vi "CSM MDI.vi"(7 "Name (\"\" to Use UUID)":string="Event CSM") -> ()   [LabVIEW 2020, in "MDI ViewManager.lvlib"]
uses:
  MDI ViewManager.lvlib
  Typedef/View.ctl
  <vilib>/Utility/miscctls.llb/LVPointTypeDef.ctl
  <vilib>/Utility/miscctls.llb/LVPoint32TypeDef.ctl
  Typedef/Layout.ctl
  <vilib>/Utility/miscctls.llb/LVBoundsTypeDef.ctl
  <vilib>/Utility/miscctls.llb/LVPositionTypeDef.ctl
  <vilib>/Utility/miscctls.llb/LVRectTypeDef.ctl
  Typedef/Update View.ctl
  49dae65a-a1df-4644-8631-e10cd2ecf887.vi
  81b46446-0aca-48f9-86dc-ebdbbb8ef4b6.vi
  7ba8cf38-d999-4af7-9cb2-e6092c4454ab.vi
  5110686f-90b8-48a6-8112-abce107b1655.vi
  <userlib>/_NEVSTOP/Communicable State Machine(CSM)/AdvanceAPI/CSM - Revert Arguments-Safe String.vi
  <userlib>/_NEVSTOP/Communicable State Machine(CSM)/_Shared/Trim Single-line Text.vi
  <userlib>/_NEVSTOP/Communicable State Machine(CSM)/AdvanceAPI/CSM - Make String Arguments Safe.vi
  <userlib>/_NEVSTOP/Communicable State Machine(CSM)/AdvanceAPI/CSM - Break Down Multiple States String.vi
  <userlib>/_NEVSTOP/Communicable State Machine(CSM)/AdvanceAPI/CSM - Compact Multiple States.vi
  49dae65a-a1df-4644-8631-e10cd2ecf887.vi/b09b9099-6be0-413b-8afc-4908471460c3.vi
  <userlib>/_NEVSTOP/Communicable State Machine(CSM)/addons/INI-Static-Variable-Support/_Support/FlagInstance-CSMINIVariable.vi
  81b46446-0aca-48f9-86dc-ebdbbb8ef4b6.vi/99de0c97-112a-4c86-9094-c187659127e1.vi
  <userlib>/_NEVSTOP/Communicable State Machine(CSM)/AdvanceAPI/CSM - Keywords.vi
  <userlib>/_NEVSTOP/Communicable State Machine(CSM)/_Support/ChangeFlag/ChangeFlag-Read.vi
  <userlib>/_NEVSTOP/Communicable State Machine(CSM)/_Support/ChangeFlag/ChangeFlagDB.vi
  <vilib>/Utility/Data Type/Get Type Information.vi
  <userlib>/_NEVSTOP/Communicable State Machine(CSM)/addons/API-String-Arugments-Support/_Support/Data To SingleElementsArray_csm.vi
  <userlib>/_NEVSTOP/Communicable State Machine(CSM)/addons/INI-Static-Variable-Support/_Support/Parse Used Session and Name.vi
  <userlib>/_NEVSTOP/Communicable State Machine(CSM)/addons/API-String-Arugments-Support/_Support/Data To API String Arguments.vi
  <userlib>/_NEVSTOP/Communicable State Machine(CSM)/addons/INI-Static-Variable-Support/_Support/INI-FGV(lvlibp).vi
  <userlib>/_NEVSTOP/Communicable State Machine(CSM)/addons/INI-Static-Variable-Support/_Support/Populate String with INI Variable.vi
  <userlib>/_NEVSTOP/Communicable State Machine(CSM)/addons/API-String-Arugments-Support/_Support/Convert API String Arguments to Data(variant).vi
  <userlib>/_NEVSTOP/Communicable State Machine(CSM)/addons/API-String-Arugments-Support/_Support/SingleElementsArray To Data_csm.vi
  <userlib>/_NEVSTOP/Communicable State Machine(CSM)/Communicable State Machine.lvlib
  <userlib>/_NEVSTOP/Communicable State Machine(CSM)/addons/INI-Static-Variable-Support/INI-Static-Variable-Support.lvlib
panel:
  in  "Tab Control 40":T1 caption="View0"
  in  "Tab Control 39":T1 caption="View1"
  in  "Tab Control 38":T1 caption="View2"
  in  "Tab Control 37":T1 caption="View3"
  in  "Tab Control 36":T1 caption="View4"
  in  "Tab Control 35":T1 caption="View5"
  in  "Tab Control 34":T1 caption="View6"
  in  "Tab Control 33":T1 caption="View7"
  in  "Tab Control 32":T1 caption="View8"
  in  "Tab Control 31":T1 caption="View9"
  in  "Tab Control 30":T1 caption="View10"
  in  "Tab Control 29":T1 caption="View11"
  in  "Tab Control 28":T1 caption="View12"
  in  "Tab Control 27":T1 caption="View13"
  in  "Tab Control 26":T1 caption="View14"
  in  "Tab Control 25":T1 caption="View15"
  in  "Tab Control 24":T1 caption="View16"
  in  "Tab Control 23":T1 caption="View17"
  in  "Tab Control 22":T1 caption="View18"
  in  "Tab Control 21":T1 caption="View19"
  in  "Tab Control 20":T1 caption="View20"
  in  "Tab Control 19":T1 caption="View21"
  in  "Tab Control 18":T1 caption="View22"
  in  "Tab Control 17":T1 caption="View23"
  in  "Tab Control 16":T1 caption="View24"
  in  "Tab Control 15":T1 caption="View25"
  in  "Tab Control 14":T1 caption="View26"
  in  "Tab Control 13":T1 caption="View27"
  in  "Tab Control 12":T1 caption="View28"
  in  "Tab Control 11":T1 caption="View29"
  in  "Tab Control 10":T1 caption="View30"
  in  "Tab Control 9":T1 caption="View31"
  in  "Tab Control 8":T1 caption="View32"
  in  "Tab Control 7":T1 caption="View33"
  in  "Tab Control 6":T1 caption="View34"
  in  "Tab Control 5":T1 caption="View35"
  in  "Tab Control 4":T1 caption="View36"
  in  "Tab Control 3":T1 caption="View37"
  in  "Tab Control 2":T1 caption="View38"
  in  "Tab Control":T1 caption="View39"
  out "State History":string
types:
  T1 = typedef "MDI ViewManager.lvlib/View.ctl" = enum32{"Page 1", "Page 2"}
  T2 = typedef "LVPointTypeDef.ctl" = cluster{"Horizontal":i16, "Vertical":i16}
  T3 = typedef "LVPoint32TypeDef.ctl" = cluster{"Horizontal":i32, "Vertical":i32}
  T4 = typedef "MDI ViewManager.lvlib/Layout.ctl" = cluster{"Origin":T2, "Layout":cluster{"Pane Dimension":T5, "Position":T6, "Label":string, "Visible":bool, "InsertedViewName":string}[], "Horizontal Scrollbar Visibility":enum16{"Always On", "Always Off", "Off While Running"}, "Vertical Scrollbar Visibility":enum16{"Always On", "Always Off", "Off While Running"}, "Position":T6, "Rect":T7}
  T5 = typedef "LVBoundsTypeDef.ctl" = cluster{"Width":u32, "Height":u32}
  T6 = typedef "LVPositionTypeDef.ctl" = cluster{"Left":i32, "Top":i32}
  T7 = typedef "LVRectTypeDef.ctl" = cluster{"Left":i16, "Top":i16, "Right":i16, "Bottom":i16}
  T8 = typedef "MDI ViewManager.lvlib/Update View.ctl" = cluster{"Name":string, "VIPath":path, "Height(Default)":u32, "Widht(Default)":u32, "VIRef":refnum<vi>}
  T9 = cluster{"Ref":cluster{"TabCtls":refnum<vi>[], "CurrMoveCtl":refnum<vi>, "Pane":refnum<vi>, "SubPanel":refnum<vi>, "Caller VI":refnum<vi>}, "Val":cluster{"TabCtlMove?":bool, "MouseOffset":T3, "LayoutMap":map{string, T4}, "ViewMap":map{string, T8}, "Edit Mode?":bool}}
  T10 = cluster{"Current VI Reference":refnum<vi>, "Close Panel on Exit?":bool}
  T11 = cluster{"Core":cluster{"Current VI Reference":refnum<vi>, "Close Panel on Exit?":bool}, "1":cluster{"Ref":cluster{"TabCtls":refnum<vi>[], "CurrMoveCtl":refnum<vi>, "Pane":refnum<vi>, "SubPanel":refnum<vi>, "Caller VI":refnum<vi>}, "Val":cluster{"TabCtlMove?":bool, "MouseOffset":T3, "LayoutMap":map{string, T4}, "ViewMap":map{string, T8}, "Edit Mode?":bool}}}
  T12 = enum16{"Always On", "Always Off", "Off While Running"}
  T13 = enum32{"Invalid", "Standard", "Closed", "Hidden", "Minimized", "Maximized"}
  T14 = enum32{"invalid app kind", "Development System", "Run Time System", "Student Edition", "Embedded LabVIEW", "Evaluation", "Custom"}
  T15 = cluster{"TabCtl":refnum<vi>[], "Pane":refnum<vi>, "Variant":variant, "map in":map{string, T4}, "1.Ref.Caller VI":refnum<vi>}
  T16 = cluster{"Pane":refnum<vi>, "TabCtls":refnum<vi>[], "Layout Map":map{string, T4}, "View Map":map{string, T8}, "1.Ref.Caller VI":refnum<vi>}
  T17 = typedef "Communicable State Machine.lvlib/_CSM_Response Source Message.ctl" = cluster{"‘State":string, "’Arguments":string, "’Error":errorcluster}
  T18 = cluster{"TabCtlMove?":bool, "Caller VI":refnum<vi>, "CtlRef":refnum<vi>, "Double Click":bool, "Coords":T3, "Ctrl":bool}
  T19 = cluster{"CtlRef":refnum<vi>, "Coords":T3, "TabCtlMove?":bool}
  T20 = cluster{"LayoutMap":map{string, T4}, "Edit Mode?":bool}
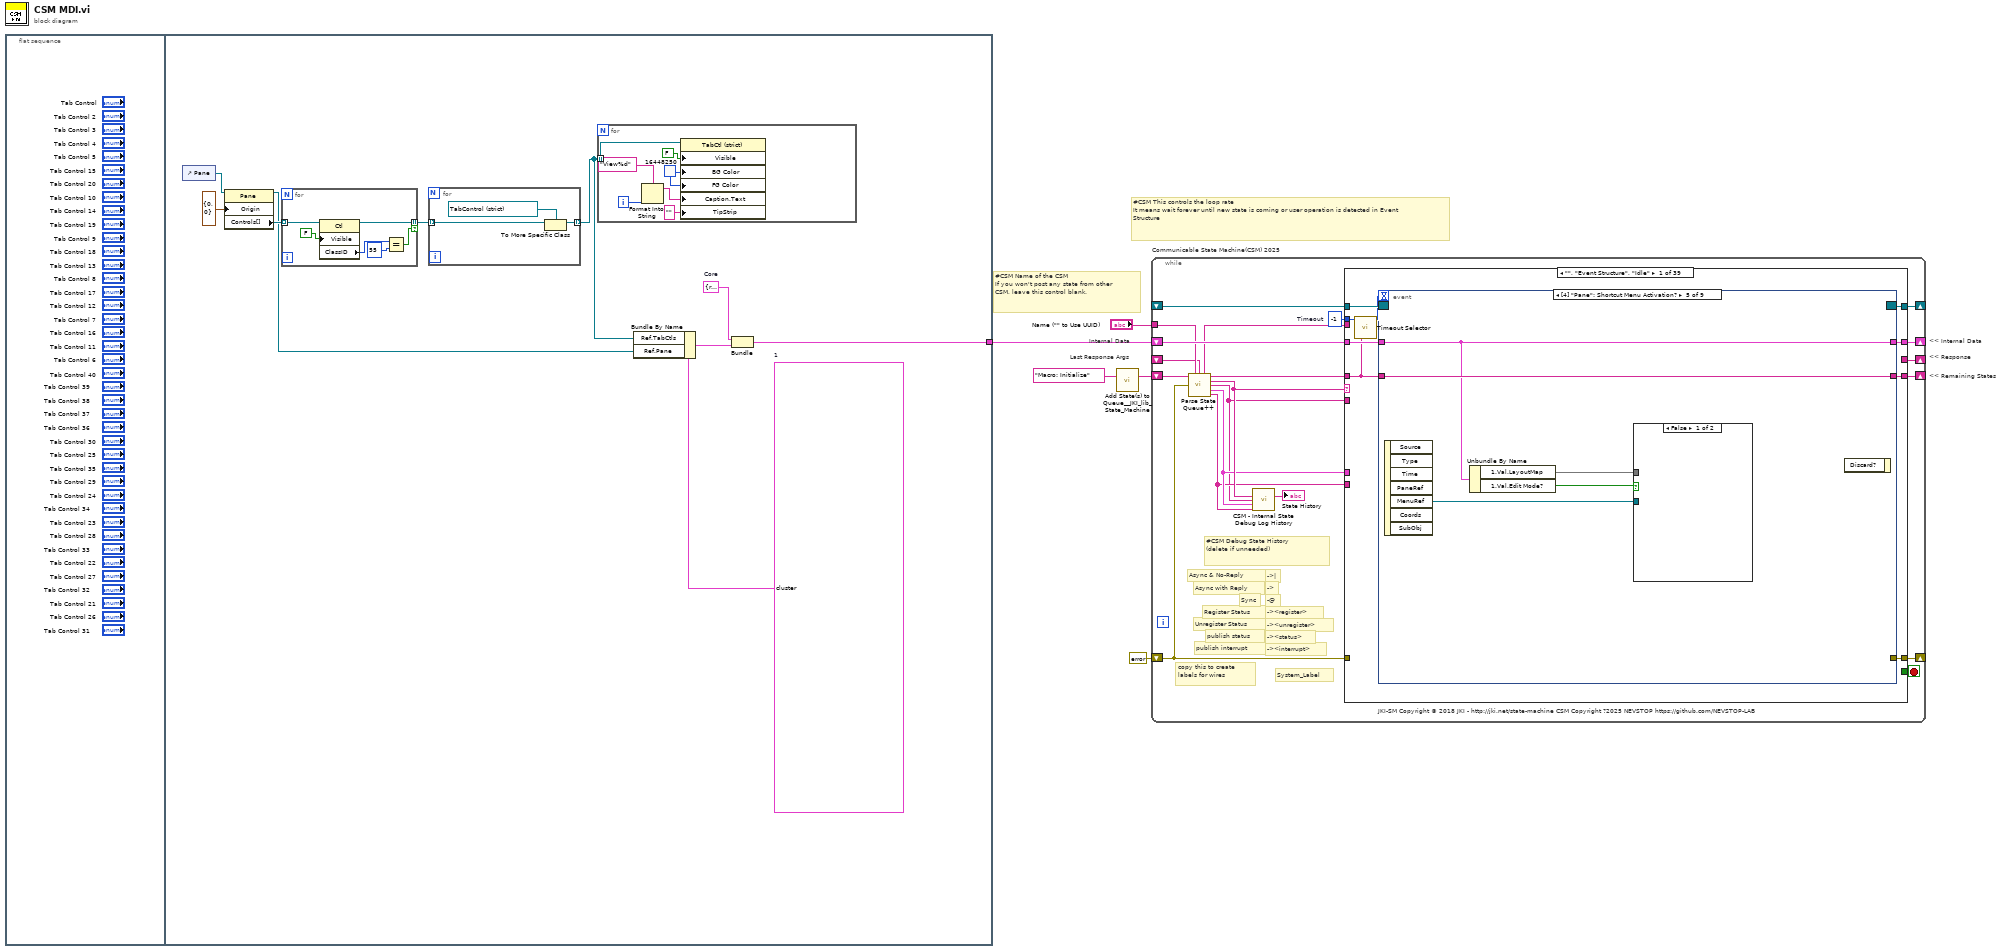
[diagram p0: block diagram]
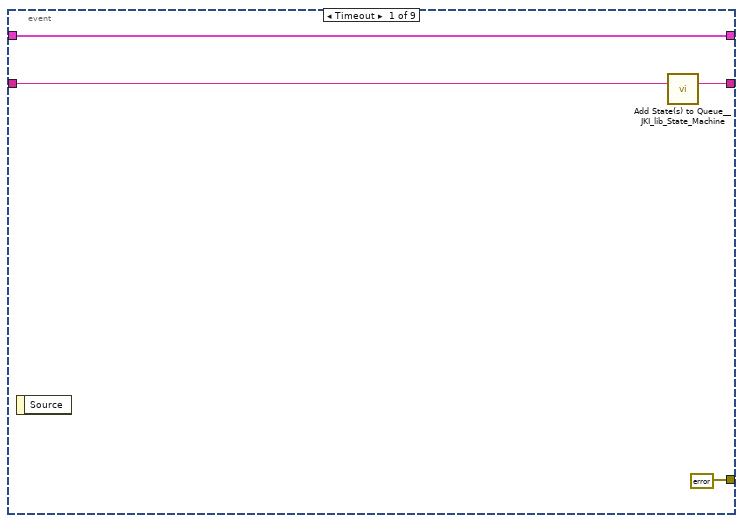
[diagram p2: hidden frame]
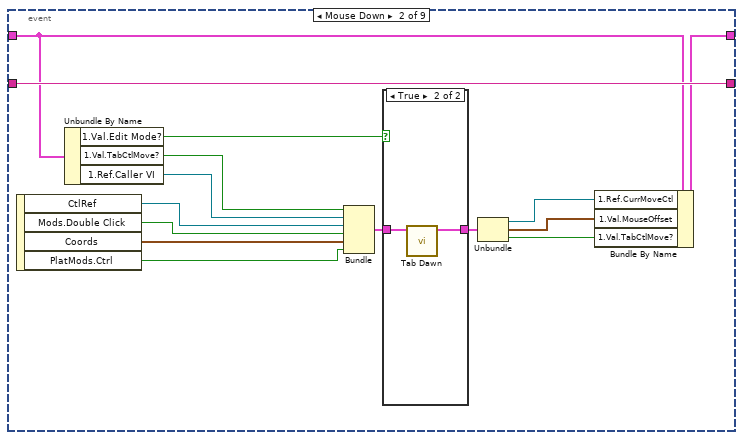
[diagram p3: hidden frame]
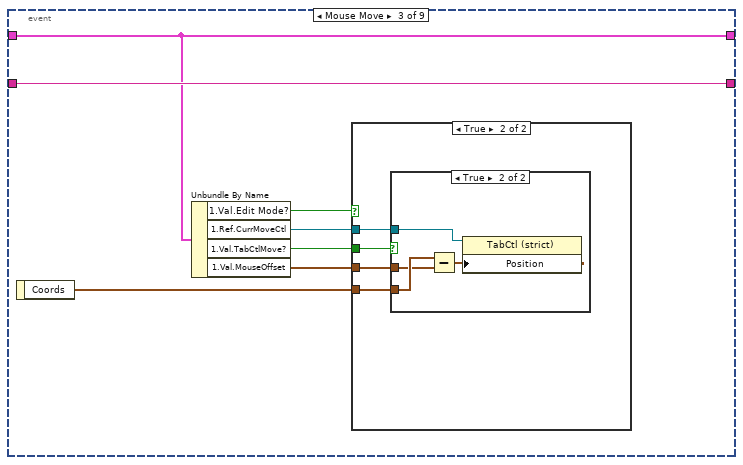
[diagram p5: hidden frame]
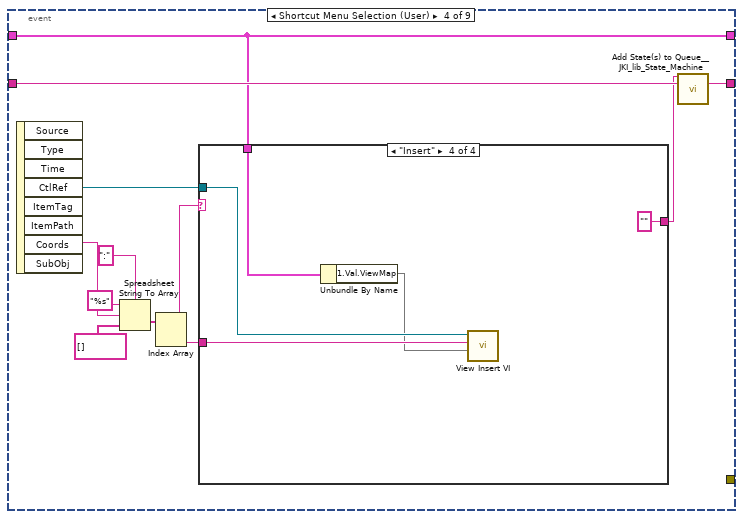
[diagram p8: hidden frame]
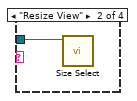
[diagram p10: hidden frame]
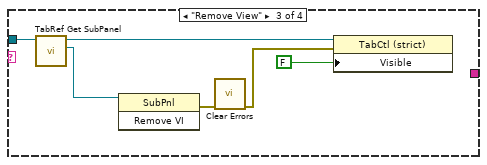
[diagram p11: hidden frame]
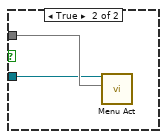
[diagram p12: hidden frame]
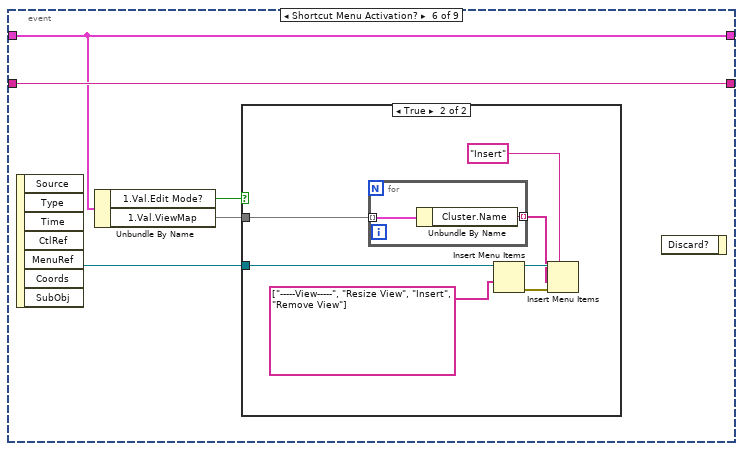
[diagram p13: hidden frame]
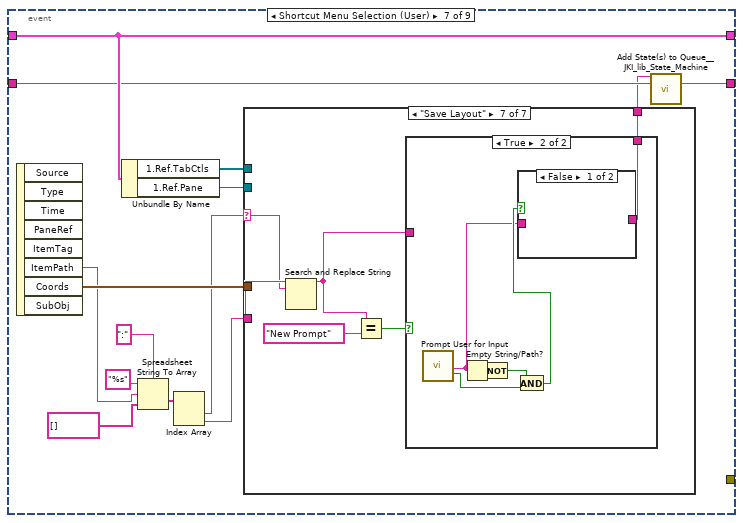
[diagram p15: hidden frame]
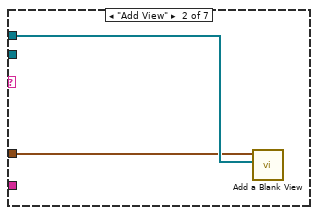
[diagram p17: hidden frame]
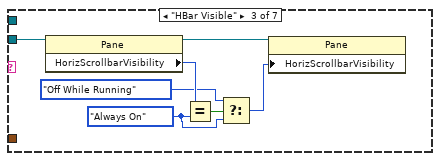
[diagram p18: hidden frame]
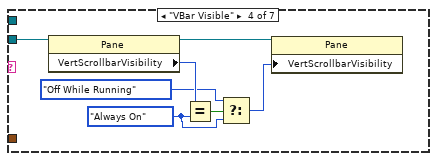
[diagram p19: hidden frame]
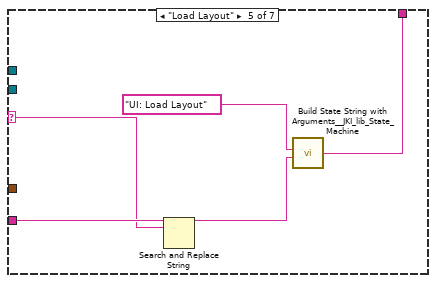
[diagram p20: hidden frame]
diagram:
  # "Last Response Args"
  # "Internal Data"
  # "<< Internal Data"
  # "<< Response"
  # "<< Remaining States"
  # "#CSM Name of the CSM\nIf you won't post any state from other CSM, leave this control blank."
  # "#CSM This controls the loop rate\nIt means wait forever until new state is coming or user operation is detected in Event Structure"
  n1 = flat-sequence {
    tunnel: [w15] -> w1
    frame #0 {
    }
    frame #1 {
      w13 = T9 {"Ref"={"TabCtls"=[], "CurrMoveCtl"=refnum, "Pane"=refnum, "SubPanel"=refnum, "Caller VI"=refnum}, "Val"={"TabCtlMove?"=FALSE, "MouseOffset"={"Horizontal"=0, "Vertical"=0}, "LayoutMap"={}, "ViewMap"={}, "Edit Mode?"=FALSE}}  # 1
      w12 = T10 {"Current VI Reference"=refnum, "Close Panel on Exit?"=FALSE}  # Core
      n2 = control-ref of="Pane"() -> (w6:refnum<vi>)
      n3 = property class="Pane"(reference=w6, "Origin"=T2 {"Horizontal"=0, "Vertical"=0}) -> (reference out=w7:refnum<vi>, "Controls[]"=w10:refnum<vi>[])  [unwired: 1 in, 1 out]
      n4 = for {
        tunnel: w10 -> [w24] mode=indexing
        tunnel: [w19] -> w9 mode=indexing if=w20
        n5 = property class="Ctl"(reference=w24, "Visible"=FALSE) -> (reference out=w19:refnum<vi>, "ClassID"=w22:u32)  [unwired: 1 in, 1 out]
        n6 = Equal?(x=w22, y=u32 55) -> (x = y?=w20:bool)
      }
      n7 = for {
        tunnel: w9 -> [w18] mode=indexing
        tunnel: [w17] -> w8 mode=indexing
        n8 = To More Specific Class(target class=refnum<vi> refnum ("Tab Control"), reference=w18) -> (specific class reference=w17:refnum<vi>)  [unwired: 1 in, 1 out]
      }
      n9 = for {
        tunnel: w8 -> [w30] mode=indexing
        i -> [w28]
        w29 = u32 16448250 ("Colors:BG Color")
        n10 = Format Into String(format string="View%d", w28) -> (resulting string=w27:string)  [unwired: 2 in, 1 out]
        n11 = property class="TabCtl (strict)"(reference=w30, "Visible"=FALSE, "BG Color"=w29, "FG Color"=w29, "Caption.Text"=w27, "TipStrip"="" ("Tip Strip")) -> ()  [unwired: 1 in, 2 out]
      }
      n12 = Bundle By Name(cluster=w13, "Ref.TabCtls"=w8, "Ref.Pane"=w7) -> (w14:T9)
      n13 = Bundle("Core"=w12, "1"=w14) -> (w15:T11)  [unwired: 1 in]
    }
  }
  n14 = call <vilib>:"Add State(s) to Queue__JKI_lib_State_Machine.vi"("State(s) in (\"\")"="Macro: Initialize" ("Init State(\"Macro: Initialize\")")) -> ("States Out"=w2:string)  [unwired: 14 in]
  n15 = while "Communicable State Machine(CSM) 2025" {
    shift-right: [w46] -> _
    shift-left: w1 -> [w45]
    shift-right: [w49] -> _
    shift-left: errorcluster {"status"=FALSE, "code"=0, "source"=""} ("error out") -> [w43]
    shift-right: [w48] -> _
    shift-left: w2 -> [w50]
    tunnel: "Name (\"\" to Use UUID)" -> [w39]
    shift-right: [w42] -> _
    shift-left: _ -> [w34]
    shift-right: [w41] -> _
    shift-left: _ -> [w40]
    stop <- w47 stop-if-true
    w44 = -1  # Timeout
    # "#CSM Debug State History\n(delete if unneeded)"
    # "-><interrupt>"
    # "-><status>"
    # "-><unregister>"
    # "-><register>"
    # "-@"
    # "->"
    # "->|"
    # "publish interrupt"
    # "publish status"
    # "Unregister Status"
    # "Register Status"
    # "Sync"
    # "Async with Reply"
    # "Async & No-Reply"
    # "copy this to create labels for wires"
    # "System_Label"
    # "JKI-SM Copyright © 2018 JKI - http://jki.net/state-machine CSM Copyright ?2025 NEVSTOP https://github.com/NEVSTOP-LAB"
    n16 = call <userlib>:"Parse State Queue++.vi"("State Queue"=w50, "Name (\"\" to Use UUID)"=w39, "Response Arguments"=w34, "Previous Error"=w43) -> ("Name Used"=w35:string, "Remaining States"=w51:string, "Current State"=w38:string, "Arguments"=w33:string, "Additional Information"=w37:T17, "Source CSM"=w36:string)  [unwired: 6 in]
    n17 = call <userlib>:"CSM - Internal State Debug Log History.vi"("State"=w38, "Arguments (\"\")"=w33, ">> Response Source Message >>"=w37, "Source (\"\")"=w36) -> ("Debug Log"=→"State History":string)  [unwired: 11 in]
    n18 = case shown="\"\", \"Event Structure\", \"Idle\"" w38 {
      selector: w38 -> [_ _ _ w223 _ _ _ _ _ _ _ _ _ _ _ _ _ _ _ _ _ _ _ _ _ _ _ _ _ _ _ _ _ _ _ _ _ _ _]
      tunnel: w51 -> [w53 w215 w220 w229 w235 w241 w267 w275 w282 w292 w301 w314 w319 w323 w329 w352 w356 w366 w370 w374 w378 w392 w412 w417 w428 w447 w458 w522 w535 w546 w549 w559 w561 w578 w586 w601 w606 w610 w614]
      tunnel: w33 -> [_ _ _ _ _ w239 w263 w270 w278 w286 _ _ _ _ _ _ _ _ _ _ _ w388 w407 w413 _ w443 w453 _ _ _ _ w550 w564 w579 w587 w597 _ _ _]
      tunnel: w45 -> [w59 w214 w217 w227 w234 w247 w268 w273 w280 w290 w300 w308 w317 w321 w326 w348 w354 w358 w369 w372 w375 w387 w410 w416 w429 w445 w455 w520 w523 w544 w548 w557 w572 w583 w591 w595 w604 w608 w612]
      tunnel: [w58 _ w218 w221 w236 errorcluster {"status"=FALSE, "code"=0, "source"=""} ("error out") w260 w269 w276 w289 _ _ _ _ _ w349 _ w361 w368 _ _ w389 w396 w418 w439 w444 w456 _ _ _ _ _ w563 w580 w588 w602 _ _ _] -> w49
      tunnel: w43 -> [_ _ w218 w222 w236 w245 w261 w271 w277 _ _ _ _ _ _ w345 _ _ _ _ _ w390 w401 w418 w439 _ _ _ _ _ _ _ w567 w580 w588 w602 _ _ _]
      tunnel: [w60 w215 w219 w228 w235 w243 w266 w274 w281 w293 w301 w313 w318 w322 w328 w351 w355 w366 w370 w373 w377 w392 w412 w417 w427 w446 w457 w521 w534 w545 w549 w559 w560 w577 w585 w601 w605 w609 w613] -> w48
      tunnel: [_ _ _ _ _ _ TRUE _ _ _ _ _ TRUE _ _ _ _ _ _ _ _ _ _ _ _ _ _ _ _ _ _ _ _ _ _ _ _ _ _] -> w47
      tunnel: [w57 w214 w217 w227 w234 w247 w268 w273 w280 w291 w300 w312 w317 w321 w325 w348 w354 w358 w369 w372 w375 w381 w410 w414 w429 w445 w455 w520 w523 w544 w548 w555 w570 w583 w591 w598 w604 w608 w612] -> w46
      tunnel: w44 -> [w55 _ _ _ _ _ _ _ _ _ _ _ _ _ _ _ _ _ _ _ _ _ _ _ _ _ _ _ _ _ _ _ _ _ _ _ _ _ _]
      tunnel: w36 -> [_ _ _ _ _ w238 _ _ _ w287 _ _ _ _ _ _ _ _ _ _ _ _ _ _ _ _ _ _ _ _ _ _ _ _ _ _ _ _ _]
      tunnel: w37 -> [_ _ _ _ _ w237 _ _ _ w288 _ _ _ _ _ _ _ _ _ _ _ _ _ _ _ _ _ _ _ _ _ _ _ _ _ _ _ _ _]
      tunnel: [_ _ _ "" w230 _ _ _ _ _ _ _ _ _ _ _ _ _ _ _ _ _ _ _ _ _ _ _ _ _ _ _ _ _ _ _ _ _ _] -> w42
      tunnel: [w52 w213 w216 w225 w233 w246 w264 w272 w279 w294 w299 w302 w315 w320 w327 w347 w353 w365 w367 w371 w376 w391 w411 w415 w438 w442 w452 w519 w533 w537 w547 w558 w575 w582 w590 w600 w603 w607 w611] -> w41
      tunnel: w40 -> [w56 w213 w216 w225 w233 w246 w264 w272 w279 w294 w299 w302 w315 w320 w327 w347 w353 _ w367 w371 w376 w391 w411 w415 w438 w442 w452 w519 w533 w537 w547 w558 w575 w582 w590 w600 w603 w607 w611]
      tunnel: w35 -> [_ _ _ w224 _ _ w262 _ _ _ _ _ _ _ w324 w343 _ w364 _ _ _ _ _ _ _ _ _ _ _ _ _ _ _ _ _ _ _ _ _]
      frame "", "Event Structure", "Idle" {
        n19 = call <userlib>:"Timeout Selector.vi"("Remaining States"=w53, "Timeout Expected"=w55) -> ("Timeout"=w54:i32)  [unwired: 5 in]
        n20 = event shown="[4] \"Pane\": Shortcut Menu Activation?" {
          selector: w56 -> [_ _ _ _ _ _ _ _ _]
          dyn-events: [_ _ _ _ _ _ _ _ _] -> w52
          timeout: w54 -> [_ _ _ _ _ _ _ _ _]
          tunnel: w53 -> [w64 w79 w88 w107 w125 w132 w153 w200 w212]
          tunnel: [w63 w79 w88 w106 w125 w132 w152 w200 w211] -> w60
          tunnel: w59 -> [w62 w78 w86 w97 w124 w131 w155 w201 w210]
          tunnel: [errorcluster {"status"=FALSE, "code"=0, "source"=""} ("error out") _ _ _ _ _ _ _ _] -> w58
          tunnel: [w62 w77 w86 w97 w124 w131 w155 w201 w210] -> w57
          event Timeout {
            n21 = event-data() -> ()  [unwired: 1 in, 1 out]
            n22 = call <vilib>:"Add State(s) to Queue__JKI_lib_State_Machine.vi"("State(s) in (\"\")"=w64) -> ("States Out"=w63:string)  [unwired: 14 in]
          }
          event Mouse Down {
            n23 = event-data() -> ("CtlRef"=w74:refnum<vi>, "Mods.Double Click"=w73:bool, "Coords"=w72:T3, "PlatMods.Ctrl"=w65:bool)  [unwired: 1 in]
            n24 = Unbundle By Name(w78) -> ("1.Val.Edit Mode?"=w66:bool, "1.Val.TabCtlMove?"=w76:bool, "1.Ref.Caller VI"=w75:refnum<vi>)
            n25 = Bundle("TabCtlMove?"=w76, "Caller VI"=w75, "CtlRef"=w74, "Double Click"=w73, "Coords"=w72, "Ctrl"=w65) -> (w71:T18)  [unwired: 1 in]
            n26 = case shown="True" w66 {
              tunnel: w71 -> [_ w81]
              tunnel: [_ w80] -> w70
              frame False {
              }
              frame True {
                n27 = call "Tab Dawn.vi"("output cluster"=w81) -> ("output cluster 2"=w80:T19)  [unwired: 10 in]
              }
            }
            n28 = Unbundle(w70) -> ("CtlRef"=w69:refnum<vi>, "Coords"=w68:T3, "TabCtlMove?"=w67:bool)
            n29 = Bundle By Name(cluster=w78, "1.Ref.CurrMoveCtl"=w69, "1.Val.MouseOffset"=w68, "1.Val.TabCtlMove?"=w67) -> (w77:T11)
          }
          event Mouse Move {
            n30 = event-data() -> ("Coords"=w87:T3)  [unwired: 1 in]
            n31 = Unbundle By Name(w86) -> ("1.Val.Edit Mode?"=w82:bool, "1.Ref.CurrMoveCtl"=w84:refnum<vi>, "1.Val.TabCtlMove?"=w85:bool, "1.Val.MouseOffset"=w83:T3)
            n32 = case shown="True" w82 {
              tunnel: w87 -> [_ w92]
              tunnel: w85 -> [_ w91]
              tunnel: w84 -> [_ w90]
              tunnel: w83 -> [_ w89]
              frame False {
              }
              frame True {
                n33 = case shown="True" w91 {
                  tunnel: w92 -> [_ w96]
                  tunnel: w90 -> [_ w95]
                  tunnel: w89 -> [_ w93]
                  frame False {
                  }
                  frame True {
                    n34 = Subtract(x=w96, y=w93) -> (x-y=w94:T3)
                    n35 = property class="TabCtl (strict)"(reference=w95, "Position"=w94) -> ()  [unwired: 1 in, 2 out]
                  }
                }
              }
            }
          }
          event Shortcut Menu Selection (User) {
            n36 = event-data() -> ("CtlRef"=w108:refnum<vi>, "ItemPath"=w103:string)  [unwired: 1 in, 6 out]
            n37 = Spreadsheet String To Array(delimiter (Tab)=":", format string="%s", spreadsheet string=w103, array type (2D Dbl)=string[] [] ("delimiter (Tab)")) -> (array=w100:string[])
            n38 = Index Array(array=w100) -> (element #1=w99:string, element #2=w98:string)  [unwired: 2 in]
            n39 = case shown="\"Insert\"" w99 {
              tunnel: w108 -> [_ w109 w115 w118]
              tunnel: [_ _ _ "" ("State(s) in Front (\"\")")] -> w105
              tunnel: w98 -> [_ _ _ w119]
              tunnel: w97 -> [_ _ _ w120]
              frame "False", Default {
              }
              frame "Resize View" {
                n40 = call "Size Select.vi"("CtlRef"=w109) -> ()  [unwired: 11 in]
              }
              frame "Remove View" {
                n41 = call "TabRef Get SubPanel.vi"("TabControl in"=w115) -> ("Sub Panel"=w111:refnum<vi>, "TabControl out"=w114:refnum<vi>)  [unwired: 8 in, 1 out]
                n42 = invoke class="SubPnl" method="Remove VI"(reference=w111) -> (error out=w112:errorcluster)  [unwired: 2 in, 2 out]
                n43 = call <vilib>:"Clear Errors.vi"("error in (no error)"=w112) -> ("error out"=w110:errorcluster)  [unwired: 5 in, 1 out]
                n44 = property class="TabCtl (strict)"(reference=w114, error in=w110, "Visible"=FALSE) -> ()  [unwired: 2 out]
              }
              frame "Insert" {
                n45 = Unbundle By Name(w120) -> ("1.Val.ViewMap"=w116:map{string, T8})
                n46 = call "View Insert VI.vi"("ViewMap"=w116, "Name"=w119, "TabControl in"=w118) -> ()  [unwired: 7 in, 2 out]
              }
            }
            n47 = call <vilib>:"Add State(s) to Queue__JKI_lib_State_Machine.vi"("State(s) in Front (\"\")"=w105, "State(s) in (\"\")"=w107) -> ("States Out"=w106:string)  [unwired: 13 in]
          }
          event Shortcut Menu Activation? {
            n48 = event-data() -> ("MenuRef"=w122:refnum<k9>)  [unwired: 1 in, 6 out]
            n49 = Unbundle By Name(w124) -> ("1.Val.LayoutMap"=w123:map{string, T4}, "1.Val.Edit Mode?"=w121:bool)
            n50 = case shown="False" w121 {
              tunnel: w123 -> [_ w127]
              tunnel: w122 -> [_ w126]
              frame False {
              }
              frame True {
                n51 = call "Menu Act.vi"("LayoutMap"=w127, "Menu in"=w126) -> ()  [unwired: 10 in]
              }
            }
            n52 = event-data() -> ()  [unwired: 2 in, 1 out]
          }
          event Shortcut Menu Activation? {
            n53 = event-data() -> ("MenuRef"=w130:refnum<k9>)  [unwired: 1 in, 6 out]
            n54 = Unbundle By Name(w131) -> ("1.Val.Edit Mode?"=w128:bool, "1.Val.ViewMap"=w129:map{string, T8})
            n55 = case shown="True" w128 {
              tunnel: w130 -> [_ w134]
              tunnel: w129 -> [_ w133]
              frame False {
              }
              frame True {
                n56 = for {
                  tunnel: w133 -> [w141] mode=indexing
                  tunnel: [w140] -> w137 mode=indexing
                  n57 = Unbundle By Name(w141) -> ("Cluster.Name"=w140:string)
                }
                n58 = Insert Menu Items(7:string[] ["-----View-----", "Resize View", "Insert", "Remove View"] ("item names"), 9:w134) -> (0:w139:errorcluster, 3:w138:refnum<k9>)  [unwired: 4 in, 1 out]
                n59 = Insert Menu Items(5:"Insert", 6:w139, 7:w137, 9:w138) -> ()  [unwired: 2 in, 3 out]
              }
            }
            n60 = event-data() -> ()  [unwired: 2 in, 1 out]
          }
          event Shortcut Menu Selection (User) {
            n61 = event-data() -> ("ItemPath"=w143:string, "Coords"=w150:T3)  [unwired: 1 in, 6 out]
            n62 = Unbundle By Name(w155) -> ("1.Ref.TabCtls"=w154:refnum<vi>[], "1.Ref.Pane"=w142:refnum<vi>)
            n63 = Spreadsheet String To Array(delimiter (Tab)=":", format string="%s", spreadsheet string=w143, array type (2D Dbl)=string[] [] ("delimiter (Tab)")) -> (array=w147:string[])
            n64 = Index Array(array=w147) -> (element #1=w145:string, element #2=w144:string)  [unwired: 2 in]
            n65 = case shown="\"Save Layout\"" w145 {
              selector: w145 -> [_ _ _ _ w172 w177 w185]
              tunnel: w154 -> [_ w157 _ _ _ _ _]
              tunnel: w150 -> [_ w156 _ _ _ _ _]
              tunnel: [_ _ _ _ w175 w180 w187] -> w151
              tunnel: w144 -> [_ _ _ _ w174 w179 w186]
              tunnel: w142 -> [_ _ w164 w171 _ _ _]
              frame "False", Default {
              }
              frame "Add View" {
                n66 = call "Add a Blank View.vi"("TabCtls"=w157, "Coords"=w156) -> ()  [unwired: 9 in, 1 out]
              }
              frame "HBar Visible" {
                w159 = T12."Always On" ("y")
                n67 = property class="Pane"(reference=w164) -> (reference out=w163:refnum<vi>, "HorizScrollbarVisibility"=w162:T12)  [unwired: 1 in, 1 out]
                n68 = Equal?(x=w162, y=w159) -> (x = y?=w161:bool)
                n69 = Select(t=T12."Off While Running" ("y"), s=w161, f=w159) -> (s? t:f=w158:T12)
                n70 = property class="Pane"(reference=w163, "HorizScrollbarVisibility"=w158) -> ()  [unwired: 1 in, 2 out]
              }
              frame "VBar Visible" {
                w166 = T12."Always On" ("y")
                n71 = property class="Pane"(reference=w171) -> (reference out=w170:refnum<vi>, "VertScrollbarVisibility"=w169:T12)  [unwired: 1 in, 1 out]
                n72 = Equal?(x=w169, y=w166) -> (x = y?=w168:bool)
                n73 = Select(t=T12."Off While Running" ("y"), s=w168, f=w166) -> (s? t:f=w165:T12)
                n74 = property class="Pane"(reference=w170, "VertScrollbarVisibility"=w165) -> ()  [unwired: 1 in, 2 out]
              }
              frame "Load Layout" {
                n75 = Search and Replace String(input string=w174, search string=w172) -> (result string=w173:string)  [unwired: 6 in, 3 out]
                n76 = call <vilib>:"Build State String with Arguments__JKI_lib_State_Machine.vi"("Arguments (\"\")"=w173, "State"="UI: Load Layout" ("State(s) in Front (\"\")")) -> ("State with Arguments"=w175:string)  [unwired: 4 in]
              }
              frame "Delete Layout" {
                n77 = Search and Replace String(input string=w179, search string=w177) -> (result string=w178:string)  [unwired: 6 in, 3 out]
                n78 = call <vilib>:"Build State String with Arguments__JKI_lib_State_Machine.vi"("Arguments (\"\")"=w178, "State"="UI: Delete Layout" ("State(s) in Front (\"\")")) -> ("State with Arguments"=w180:string)  [unwired: 4 in]
              }
              frame "Save Layout" {
                n79 = Search and Replace String(input string=w186, search string=w185) -> (result string=w183:string)  [unwired: 6 in, 3 out]
                n80 = Equal?(x=w183, y="New Prompt") -> (x = y?=w182:bool)
                n81 = case shown="True" w182 {
                  tunnel: [w188 w196] -> w187
                  tunnel: w183 -> [w189 _]
                  frame False {
                    n82 = call <vilib>:"Build State String with Arguments__JKI_lib_State_Machine.vi"("Arguments (\"\")"=w189, "State"="UI: Save Layout" ("State(s) in Front (\"\")")) -> ("State with Arguments"=w188:string)  [unwired: 4 in]
                  }
                  frame True {
                    n83 = call "Prompt User for Input"() -> ("name"=w191:string, "OK"=w194:bool)  [unwired: 17 in, 1 out]
                    n84 = Empty String/Path?(string/path=w191) -> (empty?=w195:bool)
                    n85 = Not(x=w195) -> (.not. x?=w193:bool)
                    n86 = And(x=w193, y=w194) -> (x .and. y?=w192:bool)
                    n87 = case shown="False" w192 {
                      tunnel: [_ w198] -> w196
                      tunnel: w191 -> [_ w197]
                      frame False {
                      }
                      frame True {
                        n88 = call <vilib>:"Build State String with Arguments__JKI_lib_State_Machine.vi"("Arguments (\"\")"=w197, "State"="UI: Save Layout" ("State(s) in Front (\"\")")) -> ("State with Arguments"=w198:string)  [unwired: 4 in]
                      }
                    }
                  }
                }
              }
            }
            n89 = call <vilib>:"Add State(s) to Queue__JKI_lib_State_Machine.vi"("State(s) in Front (\"\")"=w151, "State(s) in (\"\")"=w153) -> ("States Out"=w152:string)  [unwired: 13 in]
          }
          event User Event {
            # "#CSM \"New State Notifier Event\"\nThis user event is used to break out CSM from waiting in the event structure, to process the next state from external. DO NOT place any code here unless you really need to."
            n90 = event-data() -> ()  [unwired: 1 in, 1 out]
          }
          event Panel Close? {
            # "#CSM Discard Panel Close?\nDiscard the event because we'll close the front panel ourselves in Macro: Exit"
            n91 = event-data() -> ()  [unwired: 1 in, 1 out]
            n92 = Call Chain() -> (call chain=w204:string[])
            n93 = Array Size(array=w204) -> (size(s)=w208:i32)
            n94 = Greater Or Equal?(x=w208, y=2) -> (x >= y?=w206:bool)
            n95 = Select(t="", s=w206, f="Macro: Exit") -> (s? t:f=w202:string)
            n96 = call <vilib>:"Add State(s) to Queue__JKI_lib_State_Machine.vi"("State(s) in Front (\"\")"=w202, "State(s) in (\"\")"=w212) -> ("States Out"=w211:string)  [unwired: 13 in]
            n97 = event-data("Discard?"=TRUE) -> ()  [unwired: 1 in, 1 out]
          }
        }
      }
      frame "CSM Documentation" {
        # "#CSM State Syntax\n\n// Comment line, all text to the right of “//” will be ignored\n// Local Message Example\nDoSth: DoA >> Arguments\n\n// Sync Call Example\nAPI: xxxx >> Arguments -@ TargetModule\n\n// Async Call Example\nAPI: xxxx >> Arguments -> TargetModule\n\n// Async Call without Reply Example\nAPI: xxxx >> Arguments ->| TargetModule\n\n// Broadcast normal status:\nStatus >> StatusArguments  -><status>\n\n// Broadcast Interrupt status:\nInterrupt >> StatusArguments  -><interrupt>\n\n// Register Source Module's status to Handler Module\nStatus@Source Module >> Handler Module@Handler Module -><register>\n\n// Unegister Source Module's status\nStatus@Source Module >> Handler Module -><unregister>"
        # "#CSM README FIRST\n\nCommunicable State Machine(CSM) is a LabVIEW application framework that builds upon JKI State Machine(JKISM). It follows the pattern of JKISM and extends the keywords to describe message communication between modules, including concepts such as Sync-Message, Async-Message, Subscription/Unsubscription of status - essential elements for creating reusable code modules. For more information, please visit the CSM wiki: https://nevstop-lab.github.io/CSM-Wiki/\n\nFor instructions on JKI State Machine, visit: \n    http://jki.net/state-machine/\nFor information about CSM, visit: \n    https://github.com/NEVSTOP-LAB"
        # "#CSM \"Documentation\"\nCase for holding CSM Documenation"
      }
      frame "---------- Core ----------" {
        # "#CSM \"Category Seperator\"\nDo not put any code in this frame."
        n98 = call <vilib>:"Add State(s) to Queue__JKI_lib_State_Machine.vi"("State(s) in (\"\")"=w220) -> ("States Out"=w219:string)  [unwired: 14 in]
      }
      frame Default {
        # "#CSM \"Default\"\nthis is used to capture unhandled states and typos"
        n99 = call <userlib>:"CSM Unhandled State Error.vi"("error in (no error)"=w222, "Undefined State"=w223, "CSM Name"=w224) -> ("error out"=w221:errorcluster)  [unwired: 8 in]
        n100 = call <vilib>:"Add State(s) to Queue__JKI_lib_State_Machine.vi"("State(s) in (\"\")"=w229) -> ("States Out"=w228:string)  [unwired: 14 in]
      }
      frame "VI Reference" {
        n101 = Unbundle By Name(w234) -> ("Core"=w232:T10)
        n102 = Unbundle By Name(w232) -> ("Current VI Reference"=w231:refnum<vi>)
        n103 = call <userlib>:"CSM - Convert Data to HexStr.vi"("Variant"=w231) -> ("HEX String (0-9,A-F)"=w230:string)  [unwired: 8 in]
      }
      frame "Error Handler" {
        # "#CSM Disable this error dialog if you need"
        # "#CSM \"Error Handler\"\nYou can also output any states to clean-up after errors occur"
        # "Clear error"
        n104 = case shown="Error" w245 {
          selector: w245 -> [_ w254]
          tunnel: [w252 w256] -> w242
          tunnel: w241 -> [w252 w255]
          tunnel: [w251 w254] -> w240
          tunnel: w239 -> [w253 _]
          tunnel: w238 -> [_ _]
          tunnel: w237 -> [_ _]
          frame No Error {
            n105 = call <userlib>:"CSM - Convert Argument to Error.vi"("Argument"=w253) -> ("Error"=w251:errorcluster)  [unwired: 4 in]
            n106 = flat-sequence {
              frame #0 {
                # "#CSM External Error Handler Case\nUsually, it's because This CSM register others' \"Error Occurred\" status with \"Error Handler\". If other CSM have any error, the error will be passed here for central handling."
              }
            }
          }
          frame Error {
            # "#CSM Internal Error Handler Case \nIf any error Occurred, \"Error Occurred\" \nstatus update will be broadcasted to system.\nParameter is Error Cluster."
            n107 = call <userlib>:"CSM - Convert Error to Argument.vi"("Error"=w254) -> ("Argument"=w258:string)  [unwired: 4 in]
            n108 = call <vilib>:"Build State String with Arguments__JKI_lib_State_Machine.vi"("Arguments (\"\")"=w258, "State"="Error Occurred" ("Status with Arguments")) -> ("State with Arguments"=w257:string)  [unwired: 4 in]
            n109 = call <userlib>:"CSM - Broadcast Status Change.vi"("Status With Arguments"=w257, "State Queue"=w255) -> ("Remaining States"=w256:string)  [unwired: 13 in]
          }
        }
        n110 = disable-structure shown="Enabled" {
          disable-tunnel: w240 -> [w249 w250]
          frame Enabled {
            # "Unhandled Error -- Display it"
            n111 = call <vilib>:"General Error Handler.vi"("error in (no error)"=w249) -> ()  [unwired: 10 in, 5 out]
          }
          frame Disabled {
            n112 = call <vilib>:"Clear Errors.vi"("error in (no error)"=w250) -> ()  [unwired: 5 in, 2 out]
          }
        }
        n113 = call <vilib>:"Add State(s) to Queue__JKI_lib_State_Machine.vi"("State(s) in Front (\"\")"="// Post Error States", "State(s) in (\"\")"=w242) -> ("States Out"=w243:string)  [unwired: 13 in]
      }
      frame "Critical Error" {
        # "#CSM \"Critical Error\"\nWhen any un-recoverable error occurs, CSM goes into this case."
        # "#CSM Stop in Critical Error\nWhen Critical Error occurs, Stop the loop immediately. Do NOT change this unless you fully understand the impact."
        n114 = call <userlib>:"CSM Critical Error.vi"("error in (no error)"=w261, "Arugments (As Reason)"=w263, "CSM Name"=w262) -> ("error out"=w260:errorcluster)  [unwired: 8 in]
        n115 = call <vilib>:"Add State(s) to Queue__JKI_lib_State_Machine.vi"("State(s) in (\"\")"=w267) -> ("States Out"=w266:string)  [unwired: 14 in]
      }
      frame "Target Timeout Error" {
        # "#CSM \"Target Timeout Error\"\nWhen This CSM could not get the sync-call response in time, This CSM goes into this case."
        n116 = call <userlib>:"CSM Target Timeout Error.vi"("error in (no error)"=w271, "Arguments (As CSM Name)"=w270) -> ("error out"=w269:errorcluster)  [unwired: 9 in]
        n117 = call <vilib>:"Add State(s) to Queue__JKI_lib_State_Machine.vi"("State(s) in (\"\")"=w275) -> ("States Out"=w274:string)  [unwired: 14 in]
      }
      frame "Target Error" {
        # "#CSM \"Target Error\"\nWhen This CSM try to communicate with an un-existed CSM, This CSM goes into this case."
        n118 = call <userlib>:"CSM Target Error.vi"("error in (no error)"=w277, "Arguments (As CSM Name)"=w278) -> ("error out"=w276:errorcluster)  [unwired: 9 in]
        n119 = call <vilib>:"Add State(s) to Queue__JKI_lib_State_Machine.vi"("State(s) in (\"\")"=w282) -> ("States Out"=w281:string)  [unwired: 14 in]
      }
      frame "Async Response", "Response" {
        # "#CSM \"Async Response\"\nHandle Async-call Response (\"Async Response\" for ->)"
        # "#CSM \"Response\"\nHandle Sync-call Response (\"Response\" for -@)"
        n120 = Unbundle(w288) -> ("‘State"=w285:string, "’Arguments"=w284:string, "’Error"=w283:errorcluster)
        n121 = case shown="Default" w285 {
          tunnel: [w295] -> w293
          tunnel: w292 -> [w296]
          tunnel: [w298] -> w291
          tunnel: w290 -> [w298]
          tunnel: [w297] -> w289
          tunnel: w283 -> [w297]
          tunnel: w287 -> [_]
          tunnel: w286 -> [_]
          tunnel: w284 -> [_]
          frame Default {
            # "#CSM Response Comments\nAfter Message is executed, CSM goes to this state for receive the response.\n    For Async Message(->), \"Async Response\" is used. This CSM will goes to \"Async Message Posted\" immediately and receive the \"Async Response\" after the callee finishes the message.\n    For Sync Message(@),  This CSM will wait until the message is done and immediately goes to \"Response\""
            n122 = call <vilib>:"Add State(s) to Queue__JKI_lib_State_Machine.vi"("State(s) in (\"\")"=w296) -> ("States Out"=w295:string)  [unwired: 14 in]
          }
        }
      }
      frame "Async Message Posted" {
        # "#CSM \"Async Message Posted\"\nAfter Async Message is posted (-> or ->| ), CSM goes to this state for post-action.\nYou can use Argument - State to tell which Async Message is called."
      }
      frame "Initialize Core Data" {
        # "#CSM \"Initialize Core Data\"\nThis is used to determine panel behavior on exit"
        # "originally closed?"
        # "exe?"
        # "If panel starts closed or is an EXE, then close it when we exit"
        n123 = property class="VI"() -> ("FP.State"=w305:T13)  [unwired: 2 in, 2 out]
        n124 = property class="App"() -> ("App.Kind"=w311:T14)  [unwired: 2 in, 2 out]
        n125 = control-ref of="Current VI Reference"() -> (w306:refnum<vi>)
        n126 = Equal?(x=w305, y=T13."Closed" ("Front Panel Window:State")) -> (x = y?=w303:bool)
        n127 = Equal?(x=w311, y=T14."Run Time System" ("Application:Kind")) -> (x = y?=w309:bool)
        n128 = Or(x=w303, y=w309) -> (x .or. y?=w307:bool)
        n129 = Bundle By Name(cluster=w308, "Core.Current VI Reference"=w306, "Core.Close Panel on Exit?"=w307) -> (w312:T11)
        n130 = call <vilib>:"Add State(s) to Queue__JKI_lib_State_Machine.vi"("State(s) in (\"\")"=w314) -> ("States Out"=w313:string)  [unwired: 14 in]
      }
      frame "Exit" {
        # "#CSM \"Exit\"\nCase for exiting the loop. No errors that occur here will be handled."
        n131 = call <vilib>:"Add State(s) to Queue__JKI_lib_State_Machine.vi"("State(s) in (\"\")"=w319) -> ("States Out"=w318:string)  [unwired: 14 in]
      }
      frame "---------- Data ----------" {
        # "#CSM \"Category Seperator\"\nDo not put any code in this frame."
        n132 = call <vilib>:"Add State(s) to Queue__JKI_lib_State_Machine.vi"("State(s) in (\"\")"=w323) -> ("States Out"=w322:string)  [unwired: 14 in]
      }
      frame "Data: Initialize" {
        n133 = in-place {
          in-place-border: w324 -> [w337]
          n134 = in-place-cluster #1(w326) -> ("1.Val.LayoutMap"=w335:map{string, T4}, "1.Val.Edit Mode?"=w334:bool)
          n135 = Bundle("LayoutMap"=w335, "Edit Mode?"=w334) -> (w333:T20)  [unwired: 1 in]
          n136 = call "CSM - Read Configuration Variable.vim"("Write If not found? (F)"=TRUE, "Section Name (\"\" as Default)"=w337, "Configuration Prototype (Cluster Prefered)"=w333) -> ("Configuration"=w332:T20)  [unwired: 5 in, 1 out]
          n137 = Unbundle(w332) -> ("LayoutMap"=w331:map{string, T4}, "Edit Mode?"=w330:bool)
          n138 = in-place-cluster #1("1.Val.LayoutMap"=w331, "1.Val.Edit Mode?"=w330) -> (w325:T11)
        }
        n139 = call <vilib>:"Add State(s) to Queue__JKI_lib_State_Machine.vi"("State(s) in (\"\")"=w329) -> ("States Out"=w328:string)  [unwired: 14 in]
      }
      frame "Data: Cleanup" {
        w346 = TRUE ("All Temp Variable to Default Ini(F)")
        # "#CSM \"Data: Cleanup\"\nCleanup any data and references, here.\n(this is called automatically, by the Macro: Exit)"
        n140 = Unbundle By Name(w348) -> ("Core.Current VI Reference"=w350:refnum<vi>, "1.Val.LayoutMap"=w340:map{string, T4}, "1.Val.Edit Mode?"=w339:bool)  [unwired: 1 out]
        n141 = Bundle("LayoutMap"=w340, "Edit Mode?"=w339) -> (w338:T20)  [unwired: 1 in]
        n142 = call "CSM - Write Configuration Variable.vim"("Section Name (\"\" as Default)"=w343, "error in (no error)"=w345, "Configuration"=w338) -> ("error out"=w341:errorcluster)  [unwired: 5 in, 1 out]
        n143 = Merge Errors(w341) -> (w342:errorcluster)
        n144 = call <userlib>:"CSM - Sync Configuration Variables to File.vi"("Write UnSupported Datatype?(F)"=w346, "All Temp Variable to Default Ini(F)"=w346, "error in (no error)"=w342) -> ("error out"=w344:errorcluster)  [unwired: 6 in]
        n145 = Close Reference(reference=w350, error in (no error)=w344) -> (error out=w349:errorcluster)
        n146 = call <vilib>:"Add State(s) to Queue__JKI_lib_State_Machine.vi"("State(s) in (\"\")"=w352) -> ("States Out"=w351:string)  [unwired: 14 in]
      }
      frame "---------- Events ----------" {
        # "#CSM \"Category Seperator\"\nDo not put any code in this frame."
        n147 = call <vilib>:"Add State(s) to Queue__JKI_lib_State_Machine.vi"("State(s) in (\"\")"=w356) -> ("States Out"=w355:string)  [unwired: 14 in]
      }
      frame "Events: Register" {
        w360 = cluster{"TabCtl":refnum<vi>[]} {"TabCtl"=[]}  # TabCtlEvent
        # "#CSM \"Events: Register\"\nRegister user event. New Message Event is registered to break CSM waiting in event structure by default."
        # "#CSM Register New Message Event\nRegister message event to break Waiting in Event structure."
        n148 = Unbundle By Name(w358) -> ("1.Ref.TabCtls"=w357:refnum<vi>[])
        n149 = Bundle By Name(cluster=w360, "TabCtl"=w357) -> (w359:cluster{"TabCtl":refnum<vi>[]})
        n150 = call <userlib>:"CSM - Get New State Notifier Event.vi"("Name (\"\" to Use UUID)"=w364) -> ("error out"=w362:errorcluster, "New State Notifier Event"=w363:refnum<user-event>)  [unwired: 9 in]
        n151 = register-events(error in=w362, w363, w359, w359, w359) -> (reference out=w365:refnum<event-registration>, error out=w361:errorcluster)  [unwired: 1 in]
      }
      frame "Events: Unregister" {
        # "#CSM \"Events: Unregister\"\nUnregister user event."
        n152 = Unregister For Events(event registration refnum=w367) -> (error out=w368:errorcluster)  [unwired: 1 in]
      }
      frame "---------- UI ----------" {
        # "#CSM \"Category Seperator\"\nDo not put any code in this frame."
        n153 = call <vilib>:"Add State(s) to Queue__JKI_lib_State_Machine.vi"("State(s) in (\"\")"=w374) -> ("States Out"=w373:string)  [unwired: 14 in]
      }
      frame "UI: Initialize" {
        # "#CSM \"UI: Initialize\"\nInitialize the User Interface, here.\n(this is called automatically, by the Macro: Init)"
        n154 = call <vilib>:"Add State(s) to Queue__JKI_lib_State_Machine.vi"("State(s) in (\"\")"=w378) -> ("States Out"=w377:string)  [unwired: 14 in]
      }
      frame "UI: Save Layout" {
        n155 = Unbundle By Name(w387) -> ("1.Ref.TabCtls"=w384:refnum<vi>[], "1.Ref.Pane"=w383:refnum<vi>, "1.Val.LayoutMap"=w382:map{string, T4}, "1.Ref.Caller VI"=w379:refnum<vi>)
        n156 = Bundle By Name(cluster=T15 {"TabCtl"=[], "Pane"=refnum, "Variant"=variant, "map in"={}, "1.Ref.Caller VI"=refnum} ("input cluster"), "TabCtl"=w384, "Pane"=w383, "map in"=w382, "1.Ref.Caller VI"=w379) -> (w385:T15)
        n157 = call "Save Layout.vi"("error in (no error)"=w390, "key"=w388, "input cluster"=w385) -> ("error out"=w389:errorcluster, "map out"=w380:map{string, T4})  [unwired: 7 in]
        n158 = Bundle By Name(cluster=w387, "1.Val.LayoutMap"=w380) -> (w381:T11)
      }
      frame "UI: Load Layout" {
        n159 = Unbundle By Name(w410) -> ("1.Ref.Pane"=w405:refnum<vi>, "1.Ref.TabCtls"=w409:refnum<vi>[], "1.Val.LayoutMap"=w408:map{string, T4}, "1.Val.ViewMap"=w406:map{string, T8}, "1.Ref.Caller VI"=w393:refnum<vi>)
        n160 = property class="VI"(reference=w393, error in=w401) -> (error out=w400:errorcluster, "Panel"=w404:refnum<vi>)  [unwired: 1 out]
        n161 = property class="Pnl"(reference=w404, error in=w400, "DeferPanUpdts"=TRUE ("Defer Panel Updates")) -> (reference out=w398:refnum<vi>, error out=w399:errorcluster)
        n162 = Bundle By Name(cluster=T16 {"Pane"=refnum, "TabCtls"=[], "Layout Map"={}, "View Map"={}, "1.Ref.Caller VI"=refnum} ("input cluster"), "Pane"=w405, "TabCtls"=w409, "Layout Map"=w408, "View Map"=w406, "1.Ref.Caller VI"=w393) -> (w394:T16)
        n163 = call "Load Layout By Name.vi"("error in (no error)"=w399, "key"=w407, "Cluster"=w394) -> ("error out"=w397:errorcluster)  [unwired: 8 in]
        n164 = property class="Pnl"(reference=w398, error in=w397, "DeferPanUpdts"=FALSE ("Defer Panel Updates")) -> (error out=w396:errorcluster)  [unwired: 1 out]
      }
      frame "UI: Delete Layout" {
        n165 = in-place {
          in-place-border: w413 -> [w419]
          n166 = in-place-cluster #2(w416) -> ("1.Val.LayoutMap"=w421:map{string, T4})
          n167 = Remove From Map(10:w419, 11:w421) -> (3:w420:map{string, T4})  [unwired: 2 out]
          n168 = in-place-cluster #2("1.Val.LayoutMap"=w420) -> (w414:T11)
        }
      }
      frame "UI: Add Main Layout" {
        w432 = "Main" ("element")
        n169 = Unbundle By Name(w429) -> ("1.Val.Edit Mode?"=w424:bool, "1.Ref.Caller VI"=w423:refnum<vi>, "1.Val.LayoutMap"=w437:map{string, T4})
        n170 = for {
          tunnel: w437 -> [w441] mode=indexing
          tunnel: [w440] -> w436 mode=indexing
          n171 = Unbundle(w441) -> (w440:string)  [unwired: 1 out]
        }
        n172 = property class="VI"(reference=w423, "Front Panel.Minimizeable"=TRUE ("Front Panel Window:Minimizable"), "Front Panel.Resizeable"=w424) -> ()  [unwired: 1 in, 2 out]
        n173 = Search 1D Array(1D array=w436, element=w432) -> (index of element=w435:i32)  [unwired: 1 in]
        n174 = Less Than 0?(x=w435) -> (x < 0?=w434:bool)
        n175 = invoke class="VI" method="FP.Open"(reference=w423, "State"=T13."Maximized") -> ()  [unwired: 3 in, 5 out]
        n176 = call <vilib>:"Build State String with Arguments__JKI_lib_State_Machine.vi"("Arguments (\"\")"=w432, "State"="UI: Save Layout" ("State(s) in Front (\"\")")) -> ("State with Arguments"=w431:string)  [unwired: 4 in]
        n177 = Select(t=w431, s=w434, f="") -> (s? t:f=w426:string)
        n178 = call <vilib>:"Add State(s) to Queue__JKI_lib_State_Machine.vi"("State(s) in Front (\"\")"=w426, "State(s) in (\"\")"=w428) -> ("States Out"=w427:string)  [unwired: 13 in]
      }
      frame "UI: Cursor Set" {
        # "Argument"
        # "#CSM \"UI: Cursor Set\"\nSet and Unset Cursor Busy.\n(Usage: \"UI: Cursor Set >> Busy|Idle\")"
        n179 = disable-structure shown="Default" {
          disable-tunnel: [w449 _] -> w444
          disable-tunnel: w443 -> [w448 _]
          frame condition #0 (active) {
            n180 = case shown="\"Idle\", Default" w448 {
              tunnel: [w450 w451] -> w449
              frame "Idle", Default {
                n181 = call <vilib>:"Unset Busy.vi"() -> ("error out"=w450:errorcluster)  [unwired: 11 in]
              }
              frame "Busy" {
                n182 = call <vilib>:"Set Busy.vi"() -> ("error out"=w451:errorcluster)  [unwired: 10 in, 1 out]
              }
            }
          }
          frame condition #1 {
          }
        }
        n183 = call <vilib>:"Add State(s) to Queue__JKI_lib_State_Machine.vi"("State(s) in (\"\")"=w447) -> ("States Out"=w446:string)  [unwired: 14 in]
      }
      frame "UI: Front Panel State" {
        # "Argument"
        # "#CSM \"UI: Front Panel State\"\nSet Front Panel Open or Closed\n(Usage: \"UI: Front Panel State >> Open|Close\")"
        n184 = Unbundle By Name(w455) -> ("Core.Current VI Reference"=w454:refnum<vi>)
        n185 = case shown="\"Hidden\", \"Hide\"" w453 {
          tunnel: [w465 w478 w489 w501 w513] -> w456
          tunnel: w454 -> [w464 w476 w488 w500 w512]
          frame "Open", "Standard", Default {
            w459 = T13."Standard" ("State")
            n186 = property class="VI"(reference=w464) -> (reference out=w462:refnum<vi>, error out=w463:errorcluster, "FP.State"=w461:T13)  [unwired: 1 in]
            n187 = Not Equal?(x=w461, y=w459) -> (x != y?=w460:bool)
            n188 = case shown="True" w460 {
              tunnel: [w469 w471] -> w465
              tunnel: w463 -> [w468 w471]
              tunnel: w462 -> [w467 _]
              tunnel: w459 -> [w466 _]
              frame True {
                n189 = invoke class="VI" method="FP.Open"(reference=w467, error in=w468, "Activate"=TRUE, "State"=w466) -> (error out=w469:errorcluster)  [unwired: 1 in, 4 out]
              }
              frame False {
              }
            }
          }
          frame "Close", "Closed" {
            n190 = property class="VI"(reference=w476) -> (reference out=w475:refnum<vi>, error out=w477:errorcluster, "FP.State"=w473:T13)  [unwired: 1 in]
            n191 = Not Equal?(x=w473, y=T13."Closed" ("Front Panel Window:State")) -> (x != y?=w472:bool)
            n192 = case shown="True" w472 {
              tunnel: [w479 w482] -> w478
              tunnel: w477 -> [w479 w481]
              tunnel: w475 -> [_ w480]
              frame False {
              }
              frame True {
                n193 = invoke class="VI" method="FP.Close"(reference=w480, error in=w481) -> (error out=w482:errorcluster)  [unwired: 1 in, 2 out]
              }
            }
          }
          frame "Hidden", "Hide" {
            w483 = T13."Hidden" ("State")
            n194 = property class="VI"(reference=w488) -> (reference out=w486:refnum<vi>, error out=w487:errorcluster, "FP.State"=w485:T13)  [unwired: 1 in]
            n195 = Not Equal?(x=w485, y=w483) -> (x != y?=w484:bool)
            n196 = case shown="True" w484 {
              tunnel: [w493 w494] -> w489
              tunnel: w487 -> [w492 w494]
              tunnel: w486 -> [w491 _]
              tunnel: w483 -> [w490 _]
              frame True {
                n197 = invoke class="VI" method="FP.Open"(reference=w491, error in=w492, "State"=w490) -> (error out=w493:errorcluster)  [unwired: 2 in, 4 out]
              }
              frame False {
              }
            }
          }
          frame "Minimize", "Minimized" {
            w495 = T13."Minimized" ("State")
            n198 = property class="VI"(reference=w500) -> (reference out=w498:refnum<vi>, error out=w499:errorcluster, "FP.State"=w497:T13)  [unwired: 1 in]
            n199 = Not Equal?(x=w497, y=w495) -> (x != y?=w496:bool)
            n200 = case shown="False" w496 {
              tunnel: [w505 w506] -> w501
              tunnel: w499 -> [w504 w506]
              tunnel: w498 -> [w503 _]
              tunnel: w495 -> [w502 _]
              frame True {
                n201 = invoke class="VI" method="FP.Open"(reference=w503, error in=w504, "State"=w502) -> (error out=w505:errorcluster)  [unwired: 2 in, 4 out]
              }
              frame False {
              }
            }
          }
          frame "Maximize", "Maximized" {
            w507 = T13."Maximized" ("State")
            n202 = property class="VI"(reference=w512) -> (reference out=w510:refnum<vi>, error out=w511:errorcluster, "FP.State"=w509:T13)  [unwired: 1 in]
            n203 = Not Equal?(x=w509, y=w507) -> (x != y?=w508:bool)
            n204 = case shown="True" w508 {
              tunnel: [w517 w518] -> w513
              tunnel: w511 -> [w516 w518]
              tunnel: w510 -> [w515 _]
              tunnel: w507 -> [w514 _]
              frame True {
                n205 = invoke class="VI" method="FP.Open"(reference=w515, error in=w516, "State"=w514) -> (error out=w517:errorcluster)  [unwired: 2 in, 4 out]
              }
              frame False {
              }
            }
          }
        }
        n206 = call <vilib>:"Add State(s) to Queue__JKI_lib_State_Machine.vi"("State(s) in (\"\")"=w458) -> ("States Out"=w457:string)  [unwired: 14 in]
      }
      frame "---------- Macro ----------" {
        # "#CSM \"Category Seperator\"\nDo not put any code in this frame."
        n207 = call <vilib>:"Add State(s) to Queue__JKI_lib_State_Machine.vi"("State(s) in (\"\")"=w522) -> ("States Out"=w521:string)  [unwired: 14 in]
      }
      frame "Macro: Initialize" {
        w526 = "Data: Initialize\nInitialize Core Data\nUI: Initialize\nUI: Front Panel State >> %s\nEvents: Register"  # Data: Initialize Initialize Core Data UI: Initialize UI: Front Panel State >> %s Events: Register
        # "#CSM \"Macro: Initialize\"\nInitialization Macro (This is called once, when the VI starts)"
        n208 = Call Chain() -> (call chain=w527:string[])
        n209 = Array Size(array=w527) -> (size(s)=w532:i32)
        n210 = Greater Or Equal?(x=w532, y=2) -> (x >= y?=w530:bool)
        n211 = Select(t="Hide", s=w530, f="Open") -> (s? t:f=w525:string)
        n212 = Format Into String(format string=w526, w525) -> (resulting string=w524:string)  [unwired: 2 in, 1 out]
        n213 = call <vilib>:"Add State(s) to Queue__JKI_lib_State_Machine.vi"("State(s) in Front (\"\")"=w524, "State(s) in (\"\")"=w535) -> ("States Out"=w534:string)  [unwired: 13 in]
      }
      frame "Macro: Exit" {
        # "#CSM \"Macro: Exit\"\nExit Macro (This is called once, when the VI exits)"
        n214 = Unbundle By Name(w544) -> ("Core.Close Panel on Exit?"=w543:bool)
        n215 = Select(t="UI: Front Panel State >> Close", s=w543, f="") -> (s? t:f=w540:string)
        n216 = call <vilib>:"Add State(s) to Queue__JKI_lib_State_Machine.vi"("State(s) in Front (\"\")"="//Exit Sub-Modules ", "State(s) in (\"\")"=w540, "State(s) at Back (\"\")"="Data: Cleanup\nEvents: Unregister\nExit") -> ("States Out"=w538:string)  [unwired: 12 in]
        n217 = call <vilib>:"Add State(s) to Queue__JKI_lib_State_Machine.vi"("State(s) in Front (\"\")"=w538, "State(s) in (\"\")"=w546) -> ("States Out"=w545:string)  [unwired: 13 in]
      }
      frame "---------- API ----------" {
        # "#CSM \"Category Seperator\"\nDo not put any code in this frame."
      }
      frame "API: Update View" {
        # "#CSM API Example\nCopy/Rename this case for your own API"
        n218 = call "Convert API String Arguments to Data.vim"("Reference Type"=T8 {"Name"="", "VIPath"=path "", "Height(Default)"=0, "Widht(Default)"=0, "VIRef"=refnum} ("value"), "API String"=w550) -> ("Data"=w551:T8)  [unwired: 6 in, 1 out]
        n219 = Unbundle By Name(w557) -> ("1.Val.ViewMap"=w556:map{string, T8})
        n220 = Unbundle By Name(w551) -> ("Name"=w552:string)
        n221 = Insert Into Map(map in=w556, key=w552, value=w551) -> (map out=w554:map{string, T8})  [unwired: 2 out]
        n222 = Bundle By Name(cluster=w557, "1.Val.ViewMap"=w554) -> (w555:T11)
      }
      frame "API: Update Subpanel" {
        w565 = refnum<vi> refnum  # SubPanel
        # "#CSM API Example\nCopy/Rename this case for your own API"
        n223 = Unbundle By Name(w572) -> ("Core.Current VI Reference"=w571:refnum<vi>)
        n224 = call "Convert API String Arguments to Data.vim"("Reference Type"=w565, "error in (no error)"=w567, "API String"=w564) -> ("error out"=w566:errorcluster, "Data"=w569:refnum<vi>)  [unwired: 5 in]
        n225 = property class="SubPnl"(reference=w569) -> ("OwningVI"=w568:refnum<vi>)  [unwired: 1 in, 2 out]
        n226 = invoke on="Invoke Node" class="VI" method="FP.Close"(reference=w571, error in=w566) -> (reference out=w573:refnum<vi>, error out=w574:errorcluster)  [unwired: 1 in, 1 out]
        n227 = invoke on="Invoke Node" class="SubPnl" method="Insert VI"(reference=w569, error in=w574, "VI Ref"=w573) -> (error out=w563:errorcluster)  [unwired: 1 in, 3 out]
        n228 = Bundle By Name(cluster=w572, "1.Ref.Caller VI"=w568) -> (w570:T11)
        n229 = call <vilib>:"Add State(s) to Queue__JKI_lib_State_Machine.vi"("State(s) in Front (\"\")"="UI: Add Main Layout" ("Remaining States"), "State(s) in (\"\")"=w561) -> ("States Out"=w560:string)  [unwired: 13 in]
      }
      frame "API: Load Layout" {
        n230 = call <vilib>:"Build State String with Arguments__JKI_lib_State_Machine.vi"("Arguments (\"\")"=w579, "State"="UI: Load Layout") -> ("State with Arguments"=w576:string)  [unwired: 4 in]
        n231 = call <vilib>:"Add State(s) to Queue__JKI_lib_State_Machine.vi"("State(s) in Front (\"\")"=w576, "State(s) in (\"\")"=w578) -> ("States Out"=w577:string)  [unwired: 13 in]
      }
      frame "API: Save Layout" {
        n232 = call <vilib>:"Build State String with Arguments__JKI_lib_State_Machine.vi"("Arguments (\"\")"=w587, "State"="UI: Save Layout") -> ("State with Arguments"=w584:string)  [unwired: 4 in]
        n233 = call <vilib>:"Add State(s) to Queue__JKI_lib_State_Machine.vi"("State(s) in Front (\"\")"=w584, "State(s) in (\"\")"=w586) -> ("States Out"=w585:string)  [unwired: 13 in]
      }
      frame "API: Edit Mode" {
        n234 = To Lower Case(string=w597) -> (all lower case string=w592:string)
        n235 = Equal?(x=w592, y="on") -> (x = y?=w593:bool)
        n236 = Unbundle By Name(w595) -> ("1.Ref.Caller VI"=w594:refnum<vi>)
        n237 = property class="VI"(reference=w594, "Front Panel.Minimizeable"=TRUE ("Front Panel Window:Minimizable"), "Front Panel.Resizeable"=w593, "Description"=w592) -> ()  [unwired: 1 in, 2 out]
        n238 = Bundle By Name(cluster=w595, "1.Val.Edit Mode?"=w593) -> (w598:T11)
      }
      frame "---------- Action ----------" {
        # "#CSM \"Category Seperator\"\nDo not put any code in this frame."
        n239 = call <vilib>:"Add State(s) to Queue__JKI_lib_State_Machine.vi"("State(s) in (\"\")"=w606) -> ("States Out"=w605:string)  [unwired: 14 in]
      }
      frame "Action: action1" {
        # "#CSM \"Internal State\"\nThis category is used for holding internal states"
        n240 = call <vilib>:"Add State(s) to Queue__JKI_lib_State_Machine.vi"("State(s) in (\"\")"=w610) -> ("States Out"=w609:string)  [unwired: 14 in]
      }
      frame "Action: action2" {
        # "#CSM \"Internal State\"\nThis category is used for holding internal states"
        n241 = call <vilib>:"Add State(s) to Queue__JKI_lib_State_Machine.vi"("State(s) in (\"\")"=w614) -> ("States Out"=w613:string)  [unwired: 14 in]
      }
    }
  }
